vi "Measurement UI.vi"() -> ()   [LabVIEW 2023, in "FPT_Compression UI.lvlib"]
uses:
  FPT_Compression UI.lvlib
panel:
  in  "Measurement Graph":T1(tab)
  out "General Graph 1":T2(graph)
  out "General Graph 2":T2(graph)
  out "General Graph 3":T2(graph)
  out "General Graph 4":T2(graph)
  out "General Graph 5":T2(graph)
  out "PAE@Pin(s)":string[](array[string])
  out "Gain@Pin(s)":string[](array[string])
  out "Pout@Pin(s)":string[](array[string])
  out "Pout@Pin vs Freq":dbl[][](array[numeric])
  out "PAE vs Pin per Freq":dbl[][](array[numeric])
  in  "RFSG attenuation s2p path name":string caption="RFSG ATTENUATION S2P PATH NAME"
  in  "RFmx attenuation s2p path name":string caption="RFmx ATTENUATION S2P PATH NAME"
  in  "RFSG attenuation path name":string caption="RFSG ATTENUATION PATH NAME"
  in  "RFmx attenuation path name":string caption="RFmx ATTENUATION PATH NAME"
  out "Gain vs Pin per Freq":dbl[][](array[numeric])
  out "Group B Graph":refnum<vi>[](array[refnum])
  out "Group A Graph":refnum<vi>[](array[refnum])
  in  "Power sequencing file path":string
  in  "RFSG name":string="5842_0"
  in  "RFSG attenuation mode":T3(ring)=enum."s2p File"
  in  "RFSG s2p file path":string
  in  "RFmx name":string="5842_0"
  in  "RFmx attenuation mode":T3(ring)=enum."Constant Attenuation"
  in  "RFmx s2p file path":string
  out "All Graph Refs":refnum<vi>[](array[refnum])
  out "Pout vs Pin per Freq":dbl[][](array[numeric])
  out "OPxdB vs Freq":dbl[][](array[numeric])
  out "Linear Gain vs Freq":dbl[][](array[numeric])
  out "Frequencies":string[](array[string])
  out "OPxdB(s)":string[](array[string])
  out "Linear Gain(s)":string[](array[string])
  out "Full Data per Frequency":string[][](array[string])
  out "Pin(s)":string[](array[string])
  in  "Compression_Stimulus Mode":T4(ring)
  in  "SMU name":string caption="SMU Name"
  out "Table 2 Header":string[](array[string])
  out "Table 1 Header":string[](array[string])
  out "Gain@Pin vs Freq":dbl[][](array[numeric])
  out "PAE@Pin vs Freq":dbl[][](array[numeric])
  in  "Power sequencing file validity check":bool
  out "MeasTable 1":string[][](table)
  out "MeasTable 2":string[][](table)
  in  "Mode of operation":T5(ring) caption="Configuration"
  in  "Tab Control":T6(tab)
  in  "Power sequencing file path_update":path caption="Power Sequencing File Path"
  in  "SMU channel":string caption="SMU Channel"
  in  "SMU name_update":refnum<k15> caption="SMU Name"
  in  "RFmx port":string(combo)="port2" caption="RFmx Port"
  in  "RFSG port":string(combo)="port1" caption="RFSG Port"
  in  "RFSG name_update":refnum<k15> caption="RFSG Name"
  in  "RFSG attenuation mode_tab":T3(tab)=enum."s2p File" caption="RFSG Attenuation Mode"
  in  "RFSG external attenuation (dB)":dbl caption="External Attenuation" format="%#.3fdB"
  in  "RFSG s-parameters orientation":enum32{"Port1 Towards DUT", "Port2 Towards DUT"}(ring) caption="Orientation"
  in  "RFSG s2p file path_update":path caption="S2P File Path"
  in  "RFmx attenuation mode_tab":T3(tab)=enum."s2p File" caption="RFmx Attenuation Mode"
  in  "RFmx external attenuation (dB)":dbl caption="External Attenuation" format="%#.3fdB"
  in  "RFmx s2p file path_update":path caption="S2P File Path"
  in  "RFmx s-parameters orientation":enum32{"Port1 Towards DUT", "Port2 Towards DUT"}(ring) caption="Orientation"
  in  "RFmx name_update":refnum<k15> caption="RFmx Name"
  in  "DC & RF Mode":T4(tab)
  in  "CP_CW_DC Source Delay (s)":dbl caption="DC Source Delay" format="%#ps"
  in  "CP_PRF_RFmx Trigger Delay (s)":dbl caption="RFmx Trigger Delay" format="%#ps"
  in  "CP_PRF_PRI (s)":dbl=0.001 caption="PRI" format="%#ps"
  in  "CP_PRF_RF Pulse Width (s)":dbl=0.0001 caption="RF Pulse Width" format="%#ps"
  in  "CP_PRF_DC Source Delay (s)":dbl caption="DC Source Delay" format="%#ps"
  in  "PP_PRF_ON Current Limit (A)":dbl=0.2 caption="Pulse ON Current Limit" format="%#pA"
  in  "PP_PRF_PRI (s)":dbl=0.001 caption="PRI" format="%#ps"
  in  "PP_PRF_RF Pulse Width (s)":dbl=0.0001 caption="RF Pulse Width" format="%#ps"
  in  "PP_PRF_DC Source Delay (s)":dbl caption="DC Source Delay" format="%#ps"
  in  "PP_PRF_RFmx Trigger Delay (s)":dbl caption="RFmx Trigger Delay" format="%#ps"
  in  "PP_PRF_DC Pulse Width (s)":dbl=0.0008 caption="DC Pulse Width" format="%#ps"
  in  "PP_PRF_Bias Voltage Level (V)":dbl caption="Pulse OFF Voltage Level" format="%#pV"
  in  "PP_PRF_Bias Current Limit (A)":dbl=0.2 caption="Pulse OFF Current Limit" format="%#pA"
  in  "Compression_DC Measurement Interval (s)":dbl=5e-05 caption="DC Measurement Interval" format="%#ps"
  in  "Compression_RF Measurement Interval (s)":dbl=5e-05 caption="RF Measurement Interval" format="%#ps"
  in  "Compression_Target Pin (dBm)":dbl=1.0 caption="Target Pin" format="%#pdBm"
  in  "Compression_Expected DUT Gain (dB)":dbl=17.5 caption="Expected DUT Gain" format="%#pdB"
  in  "Compression_Max Linear Range (dBm)":dbl=-10.0 caption="Max Linear Range" format="%#pdBm"
  in  "Compression_Compression Point (dB)":dbl=1.0 caption="PxdB" format="%#pdB"
  in  "Compression_RFSG Frequency Start (Hz)":dbl=6000000000.0 caption="Frequency Start" step=1000000.0 format="%#pHz"
  in  "Compression_RFSG Power Start (dBm)":dbl=-20.0 caption="Power Start" format="%#pdBm"
  in  "Compression_RFSG Power Step Size (dB)":dbl=1.0 caption="Power Step Size" format="%#pdB"
  in  "Compression_RFSG Power Stop(dBm)":dbl=4.0 caption="Power End" format="%#pdBm"
  in  "Compression_RBW (Hz)":dbl=5000000.0 caption="RBW" format="%#pHz"
  in  "Compression_RFSG Frequency Stop (Hz)":dbl=18000000000.0 caption="Frequency Stop" step=1000000.0 format="%#pHz"
  in  "Compression_RFSG Number of Frequency Step":i32=10 caption="Number of Steps"
  out "Status":string
  # "Frequency Sweep"
  # "Power Sweep"
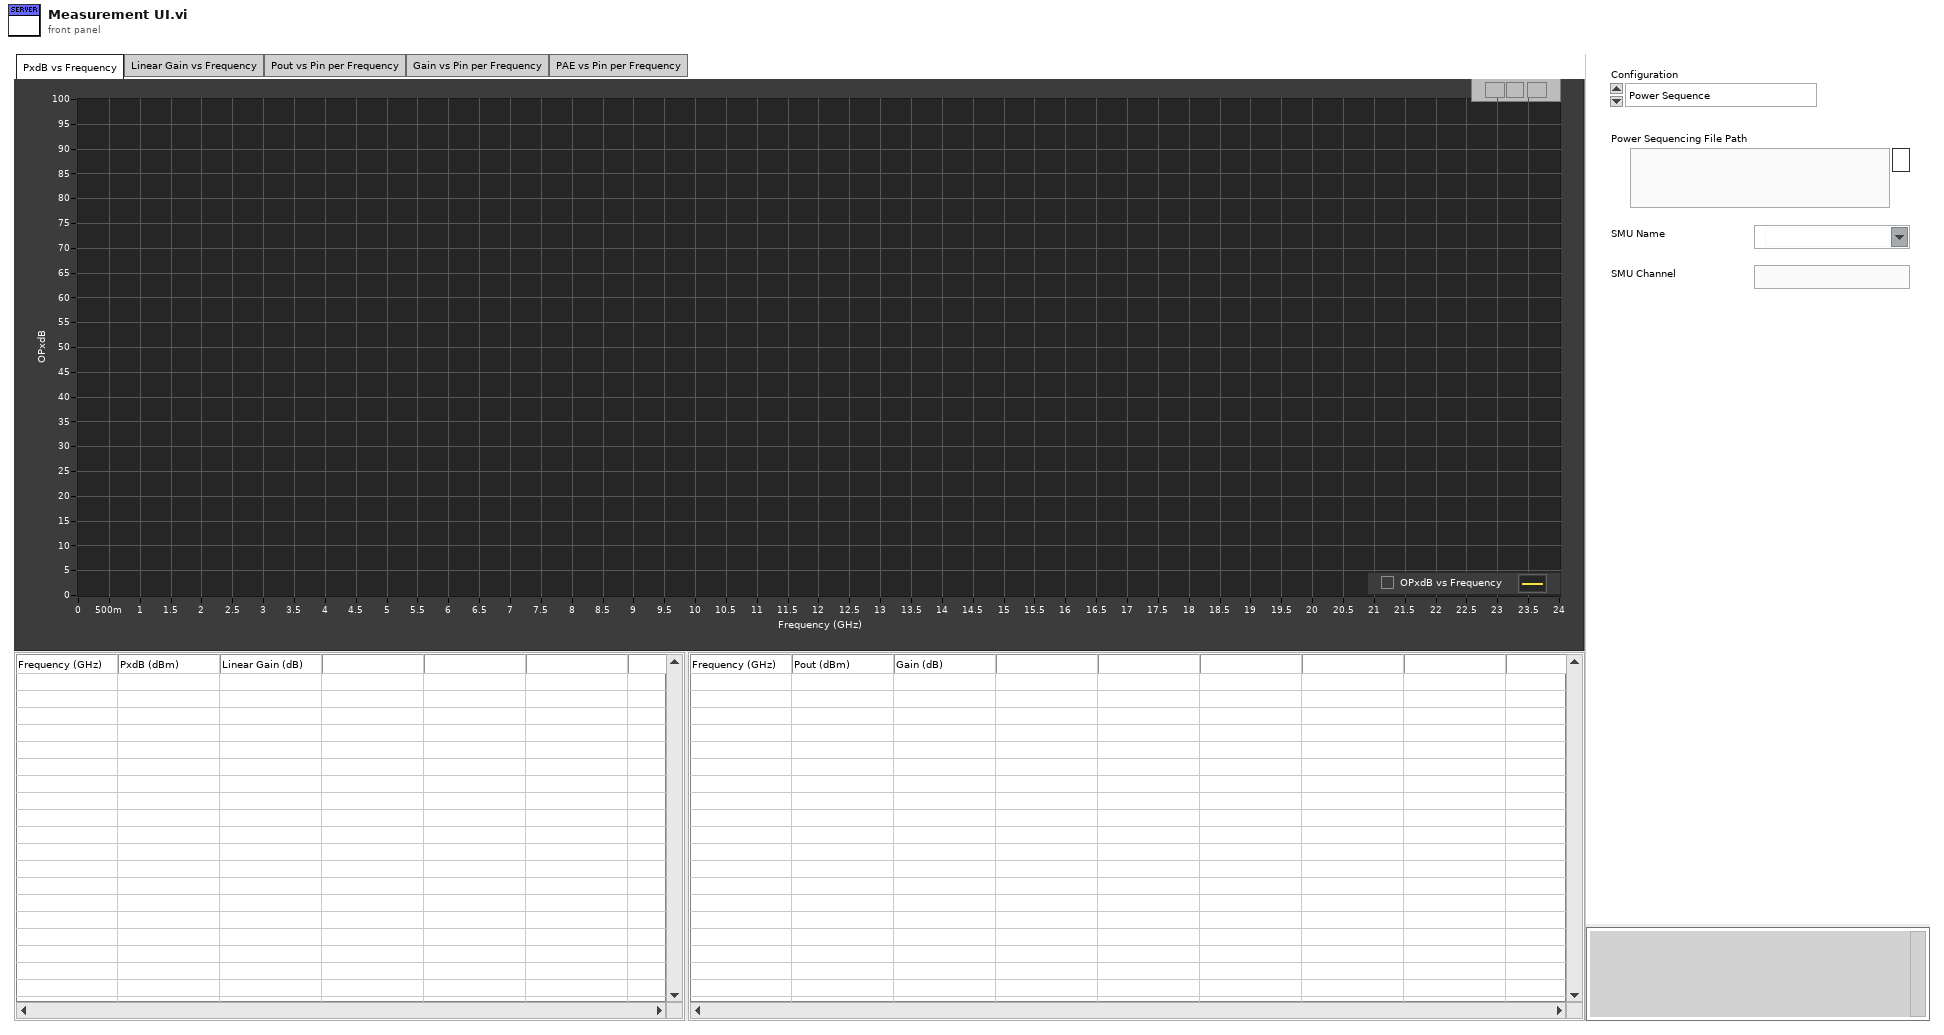
[diagram p1: front panel]
types:
  T1 = enum32{"PxdB vs Frequency", "Linear Gain vs Frequency", "Pout vs Pin per Frequency", "Gain vs Pin per Frequency", "PAE vs Pin per Frequency", "Hidden Controls"}
  T2 = cluster{"Load currents":dbl[], "Efficiency":dbl[]}[]
  T3 = enum32{"<None>", "Constant Attenuation", "s2p File"}
  T4 = enum32{"Constant Power and RF", "Constant Power and Pulsed RF", "Pulsed Power and RF"}
  T5 = enum32{"Power Sequence", "HW + Correction", "Mode", "Measurement 1"}
  T6 = enum32{"Power Sequence", "Correction", "Mode", "Measurement 1"}
  T7 = enum16{"<None>", "Constant Attenuation", "s2p File"}
  T8 = cluster{"Shift":bool, "Ctrl":bool, "Alt":bool, "Cmd":bool, "Opt":bool}
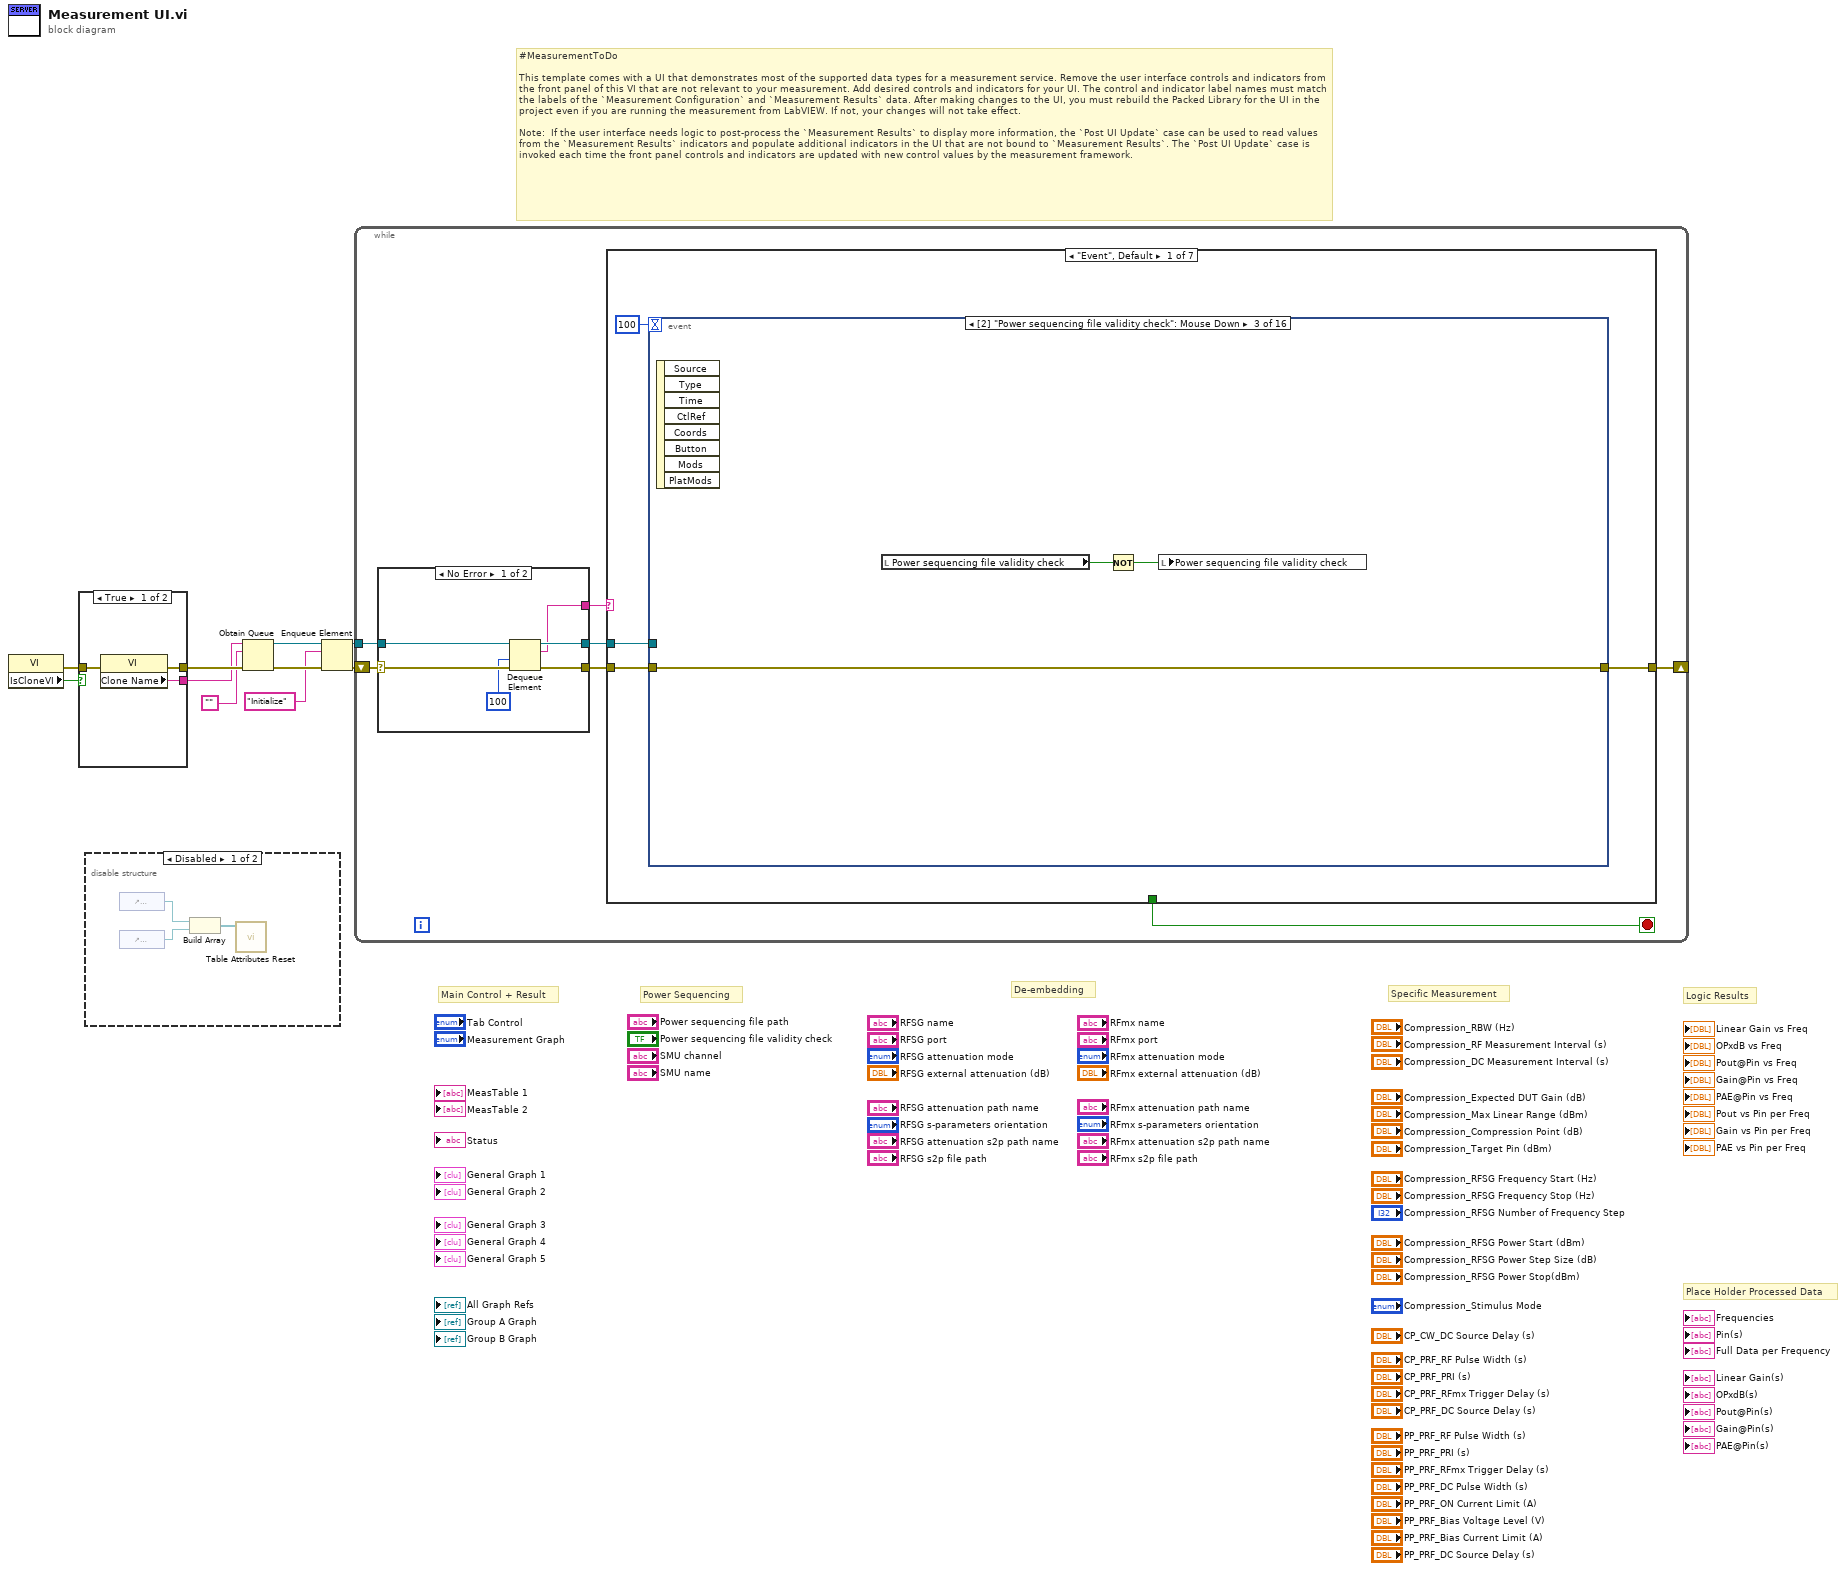
[diagram p0: block diagram]
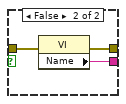
[diagram p3: hidden frame]
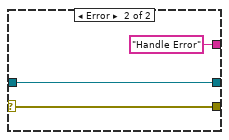
[diagram p4: hidden frame]
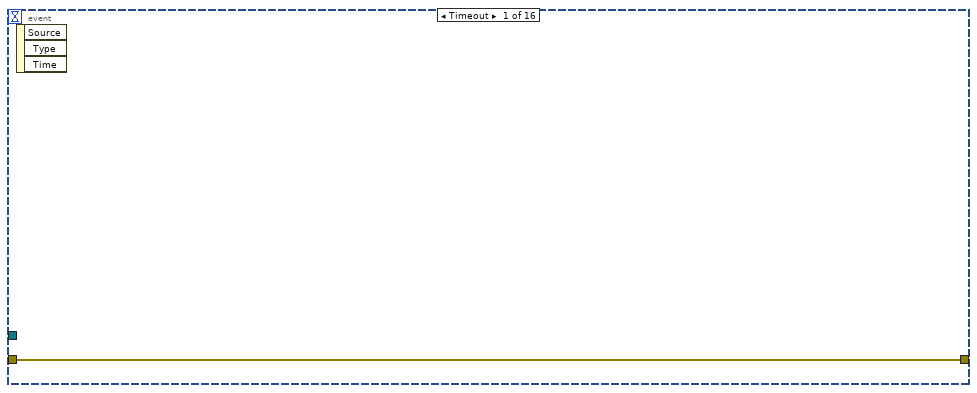
[diagram p5: hidden frame]
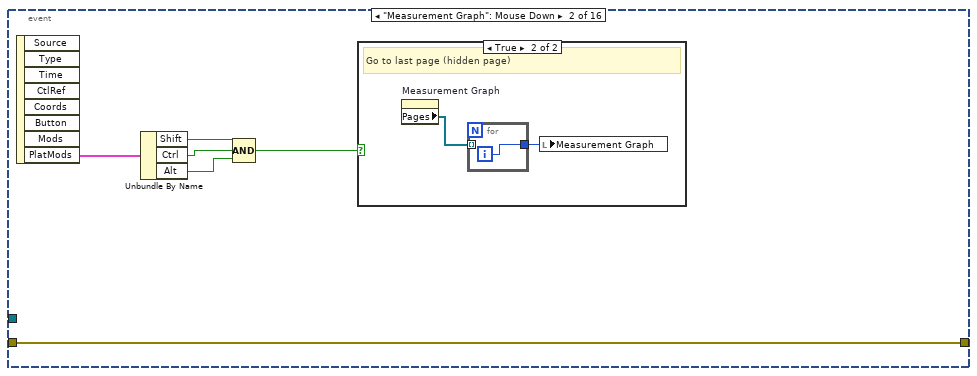
[diagram p6: hidden frame]
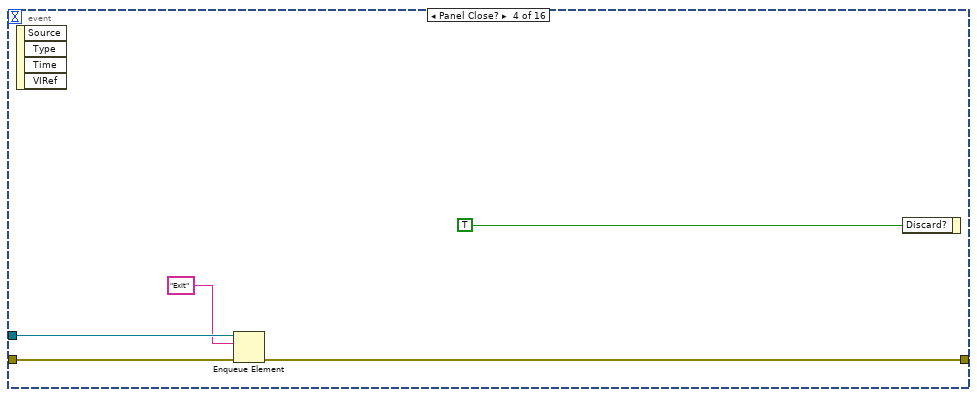
[diagram p8: hidden frame]
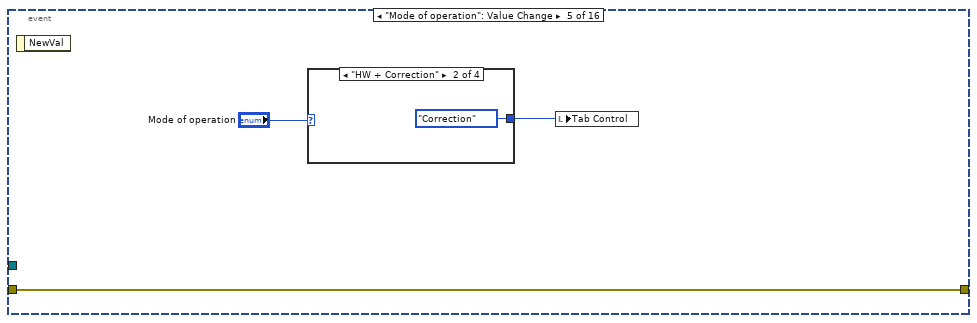
[diagram p9: hidden frame]
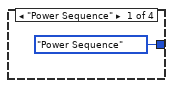
[diagram p10: hidden frame]
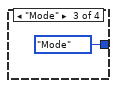
[diagram p11: hidden frame]
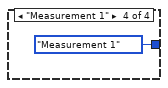
[diagram p12: hidden frame]
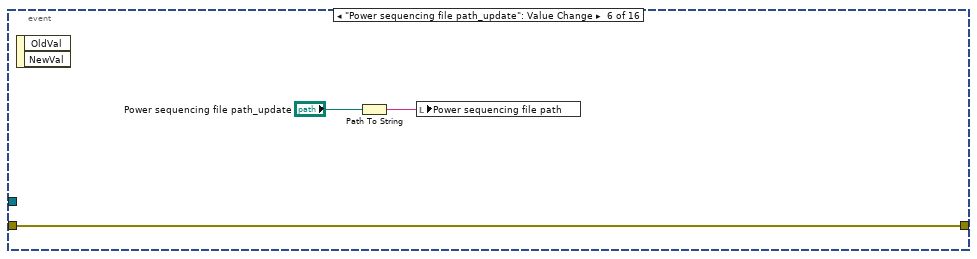
[diagram p13: hidden frame]
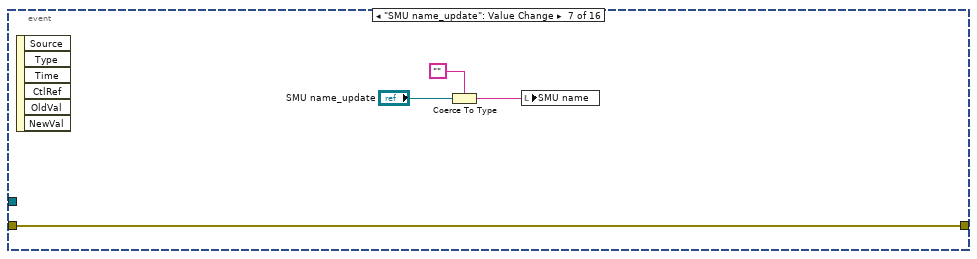
[diagram p14: hidden frame]
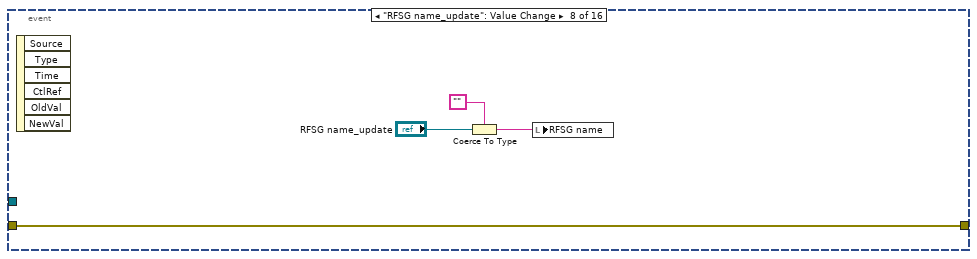
[diagram p15: hidden frame]
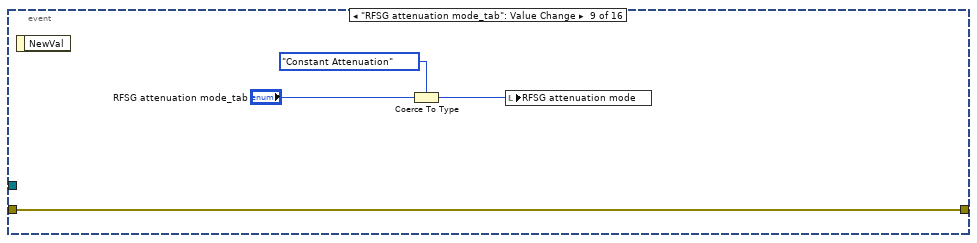
[diagram p16: hidden frame]
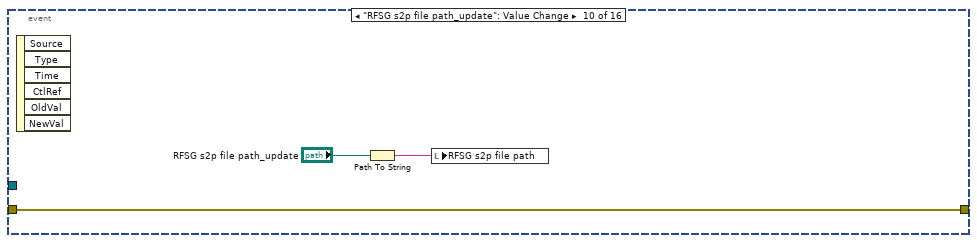
[diagram p17: hidden frame]
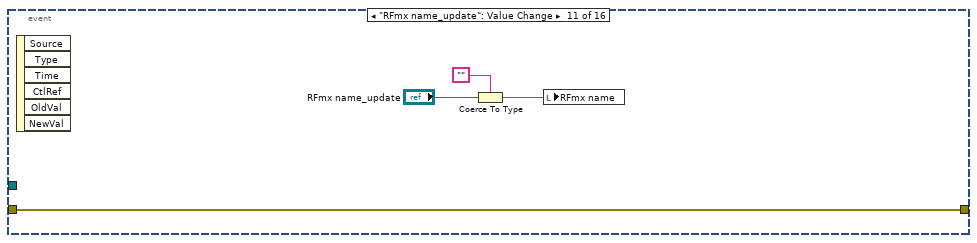
[diagram p18: hidden frame]
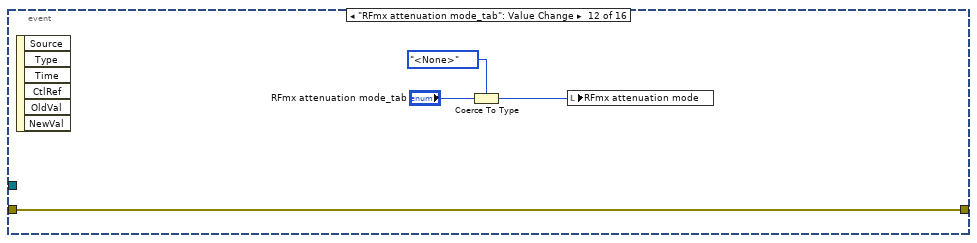
[diagram p19: hidden frame]
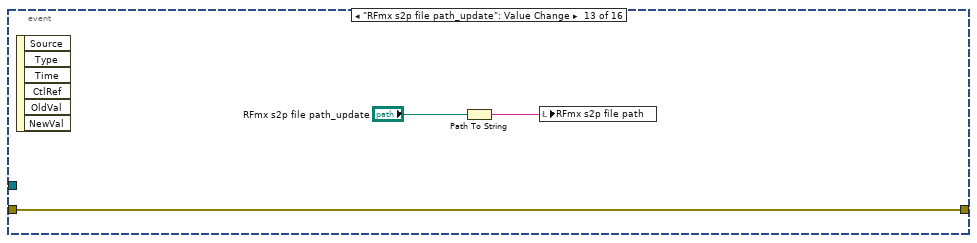
[diagram p20: hidden frame]
diagram:
  # "Logic Results"
  # "Place Holder Processed Data"
  # "Specific Measurement"
  # "De-embedding"
  # "Power Sequencing"
  # "Main Control + Result"
  # "#MeasurementToDo  \n\nThis template comes with a UI that demonstrates most of the supported data types for a measurement service. Remove the user interface controls and indicators from the front panel of this VI that are not relevant to your measurement. Add desired controls and indicators for your UI. The control and indicator label names must match the labels of the `Measurement Configuration` and `Measurement Results` data. After making changes to the UI, you must rebuild the Packed Library for the UI in the project even if you are running the measurement from LabVIEW. If not, your changes will not take effect.\n\nNote:  If the user interface needs logic to post-process the `Measurement Results` to display more information, the `Post UI Update` case can be used to read values from the `Measurement Results` indicators and populate additional indicators in the UI that are not bound to `Measurement Results`. The `Post UI Update` case is invoked each time the front panel controls and indicators are updated with new control values by the measurement framework."
  n1 = property class="VI"() -> (error out=w1:errorcluster, "IsCloneVI"=w2:bool)  [unwired: 2 in, 1 out]
  n2 = case shown="True" w2 {
    tunnel: [w13 w16] -> w10
    tunnel: [w12 w15] -> w9
    tunnel: w1 -> [w11 w14]
    frame True {
      n3 = property class="VI"(error in=w11) -> (error out=w13:errorcluster, "Clone Name"=w12:string)  [unwired: 1 in, 1 out]
    }
    frame False {
      n4 = property class="VI"(error in=w14) -> (error out=w16:errorcluster, "Name"=w15:string)  [unwired: 1 in, 1 out]
    }
  }
  n5 = disable-structure shown="Disabled" {
    frame Disabled {
      n6 = control-ref of="MeasTable 2"() -> (w19:refnum<vi>)
      n7 = control-ref of="MeasTable 1"() -> (w18:refnum<vi>)
      n8 = Build Array(w19, w18) -> (w17:refnum<vi>[])
      n9 = call "Table Attributes Reset.vi"("Table Refs"=w17) -> ()  [unwired: 11 in]
    }
    frame Enabled {
    }
  }
  n10 = Obtain Queue(name (unnamed)=w9, element data type="", error in (no error)=w10) -> (queue out=w6:refnum<queue>, error out=w8:errorcluster)  [unwired: 2 in, 1 out]
  n11 = Enqueue Element(queue=w6, element="Initialize", error in (no error)=w8) -> (queue out=w5:refnum<queue>, error out=w7:errorcluster)  [unwired: 1 in, 1 out]
  n12 = while {
    shift-right: [w21] -> _
    shift-left: w7 -> [w26]
    tunnel: w5 -> [w24]
    stop <- w20 stop-if-true
    n13 = case shown="No Error" w26 {
      selector: w26 -> [w32 w35]
      tunnel: [w31 w35] -> w25
      tunnel: w24 -> [w30 w34]
      tunnel: [w29 w34] -> w23
      tunnel: [w28 "Handle Error"] -> w22
      frame No Error {
        n14 = Dequeue Element(queue=w30, timeout in ms (-1)=100, error in (no error)=w32) -> (queue out=w29:refnum<queue>, element=w28:string, error out=w31:errorcluster)  [unwired: 1 out]
      }
      frame Error {
      }
    }
    n15 = case shown="\"Event\", Default" w22 {
      tunnel: w25 -> [w38 w153 w220 w262 w270 w277 w278]
      tunnel: w23 -> [w36 _ w219 w260 _ w275 _]
      tunnel: [w39 w153 w220 w261 w265 w272 w278] -> w21
      tunnel: [_ _ _ _ _ TRUE _] -> w20
      frame "Event", Default {
        n16 = event shown="[2] \"Power sequencing file validity check\": Mouse Down" {
          selector: _ -> [_ _ _ _ _ _ _ _ _ _ _ _ _ _ _ _]
          dyn-events: _ -> [_ _ _ _ _ _ _ _ _ _ _ _ _ _ _ _]
          timeout: 100 -> [_ _ _ _ _ _ _ _ _ _ _ _ _ _ _ _]
          tunnel: [w40 w41 w52 w55 w59 w65 w71 w72 w76 w80 w83 w87 w91 w97 w110 w131] -> w39
          tunnel: w38 -> [w40 w41 w52 w56 w59 w65 w71 w72 w76 w80 w83 w87 w91 w97 w112 w132]
          tunnel: w36 -> [_ _ _ w54 _ _ _ _ _ _ _ _ _ _ _ _]
          event Timeout {
            n17 = event-data() -> ()  [unwired: 1 in, 3 out]
          }
          event "Measurement Graph": Mouse Down {
            n18 = event-data() -> ("PlatMods"=w46:T8)  [unwired: 1 in, 7 out]
            n19 = Unbundle By Name(w46) -> ("Shift"=w45:bool, "Ctrl"=w44:bool, "Alt"=w43:bool)
            n20 = Compound Arithmetic op=AND(w45, w44, w43) -> (w42:bool)
            n21 = case shown="True" w42 {
              frame False {
              }
              frame True {
                # "Go to last page (hidden page)"
                n22 = property on="Measurement Graph" class="TabCtl (strict)"() -> ("Pages"=w48:refnum<vi>[])  [unwired: 2 in, 2 out]
                n23 = for {
                  tunnel: w48 -> [_] mode=indexing
                  tunnel: [w49] -> w47
                  i -> [w49]
                }
                n24 = local write "Measurement Graph"(w47) -> ()
              }
            }
          }
          event "Power sequencing file validity check": Mouse Down {
            n25 = event-data() -> ()  [unwired: 1 in, 8 out]
            n26 = local read "Power sequencing file validity check"() -> (w51:bool)
            n27 = Not(x=w51) -> (.not. x?=w50:bool)
            n28 = local write "Power sequencing file validity check"(w50) -> ()
          }
          event Panel Close? {
            n29 = event-data() -> ()  [unwired: 1 in, 4 out]
            n30 = Enqueue Element(queue=w54, element="Exit", error in (no error)=w56) -> (error out=w55:errorcluster)  [unwired: 1 in, 2 out]
            n31 = event-data("Discard?"=TRUE) -> ()  [unwired: 1 in, 1 out]
          }
          event "Mode of operation": Value Change {
            n32 = event-data() -> ()  [unwired: 1 in, 1 out]
            n33 = case shown="\"HW + Correction\"" "Mode of operation" {
              tunnel: [T6."Power Sequence" ("Tab Control") T6."Correction" ("Tab Control") T6."Mode" ("Tab Control") T6."Measurement 1" ("Tab Control")] -> w58
              frame "Power Sequence" {
              }
              frame "HW + Correction" {
              }
              frame "Mode" {
              }
              frame "Measurement 1" {
              }
            }
            n34 = local write "Tab Control"(w58) -> ()
          }
          event "Power sequencing file path_update": Value Change {
            n35 = event-data() -> ()  [unwired: 1 in, 2 out]
            n36 = Path To String(path="Power sequencing file path_update") -> (string=w66:string)
            n37 = local write "Power sequencing file path"(w66) -> ()
          }
          event "SMU name_update": Value Change {
            n38 = event-data() -> ()  [unwired: 1 in, 6 out]
            n39 = Coerce To Type(0:"SMU name_update", 1:"") -> (2:w68:string)
            n40 = local write "SMU name"(w68) -> ()
          }
          event "RFSG name_update": Value Change {
            n41 = event-data() -> ()  [unwired: 1 in, 6 out]
            n42 = Coerce To Type(0:"RFSG name_update", 1:"") -> (2:w73:string)
            n43 = local write "RFSG name"(w73) -> ()
          }
          event "RFSG attenuation mode_tab": Value Change {
            n44 = event-data() -> ()  [unwired: 1 in, 1 out]
            n45 = Coerce To Type(0:"RFSG attenuation mode_tab", 1:T3."Constant Attenuation" ("RFSG attenuation mode")) -> (2:w78:T3)
            n46 = local write "RFSG attenuation mode"(w78) -> ()
          }
          event "RFSG s2p file path_update": Value Change {
            n47 = event-data() -> ()  [unwired: 1 in, 6 out]
            n48 = Path To String(path="RFSG s2p file path_update") -> (string=w81:string)
            n49 = local write "RFSG s2p file path"(w81) -> ()
          }
          event "RFmx name_update": Value Change {
            n50 = event-data() -> ()  [unwired: 1 in, 6 out]
            n51 = Coerce To Type(0:"RFmx name_update", 1:"") -> (2:w85:string)
            n52 = local write "RFmx name"(w85) -> ()
          }
          event "RFmx attenuation mode_tab": Value Change {
            n53 = event-data() -> ()  [unwired: 1 in, 6 out]
            n54 = Coerce To Type(0:"RFmx attenuation mode_tab", 1:T7."<None>" ("RFmx attenuation mode")) -> (2:w88:T7)
            n55 = local write "RFmx attenuation mode"(w88) -> ()
          }
          event "RFmx s2p file path_update": Value Change {
            n56 = event-data() -> ()  [unwired: 1 in, 6 out]
            n57 = Path To String(path="RFmx s2p file path_update") -> (string=w92:string)
            n58 = local write "RFmx s2p file path"(w92) -> ()
          }
          event "DC & RF Mode": Value Change {
            n59 = event-data() -> ()  [unwired: 1 in, 6 out]
            n60 = Coerce To Type(0:"DC & RF Mode", 1:T4."Constant Power and RF" ("Compression_Stimulus Mode")) -> (2:w95:T4)
            n61 = local write "Compression_Stimulus Mode"(w95) -> ()
          }
          event "General Graph 1", "General Graph 2": Cursor Move {
            n62 = event-data() -> ("CtlRef"=w103:refnum<vi>, "PointIdx"=w109:i32, "CursLoc"=w107:cluster{"X":dbl, "Y":dbl})  [unwired: 1 in, 6 out]
            n63 = Unbundle By Name(w107) -> ("X"=w106:dbl)
            n64 = property on="Group A Graph" class="Arr (strict)"() -> ("Value"=w104:refnum<vi>[])  [unwired: 2 in, 2 out]
            n65 = Search 1D Array(1D array=w104, element=w103) -> (index of element=w105:i32)  [unwired: 1 in]
            n66 = Delete From Array(array=w104, index=w105) -> (array with subset deleted=w102:refnum<vi>[])  [unwired: 1 in, 1 out]
            n67 = call "Graph Cursor Update.vi"("Action"=enum16{"Reset", "Update"}."Update", "error in"=w112, "New X position"=w106, "Cursor Type"=enum16{"Movable", "Fixed", "All"}."Movable", "Graph Refs in"=w102) -> ("error out"=w111:errorcluster)  [unwired: 5 in, 1 out]
            n68 = control-ref of="MeasTable 1"() -> (w99:refnum<vi>)
            n69 = call "Table Highlight.vi"("Action"=enum16{"Reset", "Highlight 1 Row"}."Highlight 1 Row", "error in"=w111, "Color Box"=u32 16776960, "Row"=w109, "Table Ref in"=w99) -> ("error out"=w110:errorcluster)  [unwired: 5 in, 1 out]
          }
          event "General Graph 3", "General Graph 4", "General Graph 5": Cursor Move {
            # "------------------------Table2------------------------\n<Freq><Pin><Pout><Gain><PAE>"
            n70 = event-data() -> ("CtlRef"=w125:refnum<vi>, "PointIdx"=w115:i32, "CursLoc"=w129:cluster{"X":dbl, "Y":dbl})  [unwired: 1 in, 6 out]
            n71 = Unbundle By Name(w129) -> ("X"=w128:dbl)
            n72 = property on="Group B Graph" class="Arr (strict)"() -> ("Value"=w126:refnum<vi>[])  [unwired: 2 in, 2 out]
            n73 = Search 1D Array(1D array=w126, element=w125) -> (index of element=w127:i32)  [unwired: 1 in]
            n74 = Delete From Array(array=w126, index=w127) -> (array with subset deleted=w124:refnum<vi>[])  [unwired: 1 in, 1 out]
            n75 = call "Graph Cursor Update.vi"("Action"=enum16{"Reset", "Update"}."Update", "error in"=w132, "New X position"=w128, "Cursor Type"=enum16{"Movable", "Fixed", "All"}."Movable", "Graph Refs in"=w124) -> ("error out"=w131:errorcluster)  [unwired: 5 in, 1 out]
            n76 = local read "Frequencies"() -> (w116:string[])
            n77 = local read "Pin(s)"() -> (w119:string[])
            n78 = Index Array(array=w119, index=w115) -> (element=w118:string)
            n79 = local read "Full Data per Frequency"() -> (w120:string[][])
            n80 = local read "Table 2 Header"() -> (w113:string[])
            n81 = for {
              tunnel: [w133] -> w117 mode=indexing
              tunnel: w118 -> [w133]
              tunnel: w116 -> [_] mode=indexing
            }
            n82 = control-ref of="MeasTable 2"() -> (w122:refnum<vi>)
            n83 = call "Get Data per Frequency at Pin Point Index.vi"("Pin Point Index"=w115, "Full Data per Freq"=w120) -> ("Focused Data"=w114:string[][])  [unwired: 9 in]
            n84 = Build Array (concatenate)(w116, w117, w114) -> (w121:string[][])
            n85 = call "Table Set Header Name and Data (String).vi"("Data"=w121, "Header"=w113, "Table Ref"=w122) -> ()  [unwired: 9 in]
          }
        }
      }
      frame "Initialize" {
        w145 = 0
        # "-------Go to Default Page/Tab-------"
        # "-------------------------Assign Graph References in Group-------------------------"
        n86 = local write "Tab Control"(w145) -> ()
        n87 = local write "Mode of operation"(w145) -> ()
        n88 = local write "Measurement Graph"(w145) -> ()
        n89 = control-ref of="General Graph 1"() -> (w148:refnum<vi>)
        n90 = control-ref of="General Graph 2"() -> (w147:refnum<vi>)
        n91 = control-ref of="General Graph 3"() -> (w146:refnum<vi>)
        n92 = control-ref of="General Graph 4"() -> (w137:refnum<vi>)
        n93 = control-ref of="General Graph 5"() -> (w136:refnum<vi>)
        n94 = Build Array(w148, w147, w146, w137, w136) -> (w144:refnum<vi>[])
        n95 = Build Array(w148, w147) -> (w143:refnum<vi>[])
        n96 = Build Array(w146, w137, w136) -> (w138:refnum<vi>[])
        n97 = local write "All Graph Refs"(w144) -> ()
        n98 = local write "Group A Graph"(w143) -> ()
        n99 = call "Graph Set Cursor Mode.vi"("Cursor Mode"=enum32{"Free-Drag", "Single-Plot", "Multi-Plot"}."Single-Plot", "Graph Refs in"=w143) -> ("Graph Refs out"=w149:refnum<vi>[])  [unwired: 8 in, 1 out]
        n100 = call "Graph Set Cursor Mode.vi"("Cursor Mode"=enum32{"Free-Drag", "Single-Plot", "Multi-Plot"}."Multi-Plot", "Graph Refs in"=w138) -> ("Graph Refs out"=w142:refnum<vi>[])  [unwired: 8 in, 1 out]
        n101 = local write "Group B Graph"(w138) -> ()
        n102 = call "Graph Cursor Update.vi"("Action"=enum16{"Reset", "Update"}."Reset", "Cursor Type"=enum16{"Movable", "Fixed", "All"}."All", "Graph Refs in"=w149) -> ()  [unwired: 7 in, 2 out]
        n103 = call "Graph Cursor Update.vi"("Action"=enum16{"Reset", "Update"}."Reset", "Cursor Type"=enum16{"Movable", "Fixed", "All"}."All", "Graph Refs in"=w142) -> ()  [unwired: 7 in, 2 out]
        "Table 2 Header" <- string[] ["Frequency (GHz)", "Pin (dBm)", "Pout (dBm)", "Gain (dB)", "PAE (%)"] ("Header")
        "Table 1 Header" <- string[] ["Frequency (GHz)", "PxdB (dBm)", "Linear Gain (dB)", "Pout@Target Pin", "Gain@Target Pin", "PAE@Target Pin"] ("Header")
      }
      frame "Post UI Update" {
        # "--------------------Get Pout@Pin--------------------"
        # "------------------Get PAE@Pin--------------------"
        # "--------------------Get Gain@Pin--------------------"
        # "------------Get Pout(s) and Gain(s) per Frequency------------"
        # "-------------------------Get Frequencies-------------------------"
        # "------------------Get Linear Gain------------------"
        # "--------------------Get OPxdB--------------------"
        # "--------------------Get Pin(s)--------------------"
        # "This case will be triggered, after framework updates the User interface with result values.\nUsed to update data type def"
        n104 = local read "Power sequencing file path"() -> (w216:string)
        n105 = local read "Compression_Stimulus Mode"() -> (w175:T4)
        n106 = local read "RFSG attenuation mode"() -> (w215:T3)
        n107 = local read "RFmx attenuation mode"() -> (w201:T3)
        n108 = local read "SMU name"() -> (w173:string)
        n109 = local read "RFSG s2p file path"() -> (w208:string)
        n110 = local read "RFmx s2p file path"() -> (w207:string)
        n111 = local read "RFSG name"() -> (w212:string)
        n112 = local read "RFmx name"() -> (w203:string)
        n113 = Enqueue Element(queue=w219, element="Post UI Update 2") -> ()  [unwired: 2 in, 3 out]
        n114 = Coerce To Type(0:w173, 1:refnum<k15> refnum ("RFSG name_update")) -> (2:w171:refnum<k15>)
        n115 = Coerce To Type(0:w175, 1:T4."Constant Power and RF" ("DC & RF Mode")) -> (2:w174:T4)
        n116 = local write "SMU name_update"(w171) -> ()
        n117 = Coerce To Type(0:w215, 1:T3."<None>" ("RFSG attenuation mode_tab")) -> (2:w214:T3)
        n118 = Coerce To Type(0:w203, 1:refnum<k15> refnum ("RFSG name_update")) -> (2:w205:refnum<k15>)
        n119 = String To Path(string=w207) -> (path=w206:path)
        n120 = Coerce To Type(0:w212, 1:refnum<k15> refnum ("RFSG name_update")) -> (2:w210:refnum<k15>)
        n121 = Coerce To Type(0:w201, 1:T3."<None>" ("RFmx attenuation mode_tab")) -> (2:w202:T3)
        n122 = String To Path(string=w216) -> (path=w217:path)
        n123 = String To Path(string=w208) -> (path=w209:path)
        n124 = local write "DC & RF Mode"(w174) -> ()
        n125 = local write "RFmx name_update"(w205) -> ()
        n126 = local write "RFmx attenuation mode_tab"(w202) -> ()
        n127 = local write "RFmx s2p file path_update"(w206) -> ()
        n128 = local write "Power sequencing file path_update"(w217) -> ()
        n129 = local write "RFSG name_update"(w210) -> ()
        n130 = local write "RFSG attenuation mode_tab"(w214) -> ()
        n131 = local write "RFSG s2p file path_update"(w209) -> ()
        n132 = local read "Pout vs Pin per Freq"() -> (w196:dbl[][])
        n133 = local read "Linear Gain vs Freq"() -> (w190:dbl[][])
        n134 = local read "OPxdB vs Freq"() -> (w192:dbl[][])
        n135 = Index Array(array=w196) -> (element=w195:dbl[])  [unwired: 2 in]
        n136 = Index Array(array=w192, index (row)=1) -> (element=w189:dbl[])  [unwired: 1 in]
        n137 = Index Array(array=w190, index (row)=1) -> (element=w187:dbl[])  [unwired: 1 in]
        n138 = local read "Gain vs Pin per Freq"() -> (w181:dbl[][])
        n139 = local read "PAE vs Pin per Freq"() -> (w167:dbl[][])
        n140 = local read "Pout vs Pin per Freq"() -> (w180:dbl[][])
        n141 = Number To Fractional String(number=w195) -> (F-format string=w194:string[])  [unwired: 3 in]
        n142 = Number To Fractional String(number=w189) -> (F-format string=w188:string[])  [unwired: 3 in]
        n143 = Number To Fractional String(number=w187) -> (F-format string=w186:string[])  [unwired: 3 in]
        n144 = local write "Pin(s)"(w194) -> ()
        n145 = local write "OPxdB(s)"(w188) -> ()
        n146 = local write "Linear Gain(s)"(w186) -> ()
        n147 = Delete From Array(array=w180, length=1, index (row)=0) -> (array with subset deleted=w182:dbl[][])  [unwired: 1 in, 1 out]
        n148 = Delete From Array(array=w181, length=1, index (row)=0) -> (array with subset deleted=w183:dbl[][])  [unwired: 1 in, 1 out]
        n149 = Delete From Array(array=w167, length=1, index (row)=0) -> (array with subset deleted=w166:dbl[][])  [unwired: 1 in, 1 out]
        n150 = local read "Linear Gain vs Freq"() -> (w199:dbl[][])
        n151 = Build Array (concatenate)(w182, w183, w166) -> (w184:dbl[][])
        n152 = local read "Pout@Pin vs Freq"() -> (w156:dbl[][])
        n153 = local read "Gain@Pin vs Freq"() -> (w159:dbl[][])
        n154 = local read "PAE@Pin vs Freq"() -> (w161:dbl[][])
        n155 = Number To Fractional String(number=w184) -> (F-format string=w185:string[][])  [unwired: 3 in]
        n156 = local write "Full Data per Frequency"(w185) -> ()
        n157 = Index Array(array=w199) -> (element=w198:dbl[])  [unwired: 2 in]
        n158 = for {
          tunnel: w198 -> [w223] mode=indexing
          tunnel: [w221] -> w197 mode=indexing
          # "Get Plot Names"
          n159 = Format Into String(format string="%.3fGHz", w223) -> (resulting string=w221:string)  [unwired: 2 in, 1 out]
        }
        n160 = Index Array(array=w156, index (row)=1) -> (element=w155:dbl[])  [unwired: 1 in]
        n161 = Index Array(array=w159, index (row)=1) -> (element=w162:dbl[])  [unwired: 1 in]
        n162 = Index Array(array=w161, index (row)=1) -> (element=w164:dbl[])  [unwired: 1 in]
        n163 = Number To Fractional String(number=w155) -> (F-format string=w154:string[])  [unwired: 3 in]
        n164 = Number To Fractional String(number=w162) -> (F-format string=w163:string[])  [unwired: 3 in]
        n165 = Number To Fractional String(number=w164) -> (F-format string=w165:string[])  [unwired: 3 in]
        n166 = local write "Pout@Pin(s)"(w154) -> ()
        n167 = local write "Gain@Pin(s)"(w163) -> ()
        n168 = local write "PAE@Pin(s)"(w165) -> ()
        n169 = local write "Frequencies"(w197) -> ()
      }
      frame "Post UI Update 2" {
        # "---------------Graph5---------------\nPAE vs Pin per Frequency"
        # "---------------Graph2---------------\nLinear Gain vs Frequency"
        # "---------------Graph1---------------\nOPxdB vs Frequency"
        # "---------------Graph4---------------\nGain vs Pin per Frequency"
        # "---------------Graph3---------------\nPout vs Pin per Frequency"
        # "------------------------Table1------------------------\nPout, Gain vs Pin per Freq Graph"
        # "------------------------Table2------------------------\n<Freq><Pin><Pout><Gain><PAE>"
        # "Table1: OPxdB, Gain vs Freq"
        # "Run after Post UI Update. Can be duplicate is need more processing.\nUtilize this case to convert the result to graph or table"
        n170 = local read "Linear Gain vs Freq"() -> (w248:dbl[][])
        n171 = local read "OPxdB vs Freq"() -> (w250:dbl[][])
        n172 = control-ref of="General Graph 1"() -> (w251:refnum<vi>)
        n173 = control-ref of="General Graph 2"() -> (w249:refnum<vi>)
        n174 = Enqueue Element(queue=w260, element="Post UI Update 3", error in (no error)=w262) -> (error out=w261:errorcluster)  [unwired: 1 in, 2 out]
        n175 = call "Graph Assign Plot Names and Data.vi"("Legend Number of Rows"=1, "X Ys Data"=w250, "Graph Ref in"=w251) -> ()  [unwired: 6 in, 3 out]
        n176 = call "Graph Assign Plot Names and Data.vi"("Legend Number of Rows"=1, "X Ys Data"=w248, "Graph Ref in"=w249) -> ()  [unwired: 6 in, 3 out]
        n177 = local read "Table 1 Header"() -> (w227:string[])
        n178 = local read "Linear Gain(s)"() -> (w242:string[])
        n179 = local read "Frequencies"() -> (w244:string[])
        n180 = local read "Pout@Pin(s)"() -> (w226:string[])
        n181 = local read "Gain@Pin(s)"() -> (w225:string[])
        n182 = local read "Pout vs Pin per Freq"() -> (w241:dbl[][])
        n183 = local read "PAE@Pin(s)"() -> (w224:string[])
        n184 = local read "Gain vs Pin per Freq"() -> (w255:dbl[][])
        n185 = local read "OPxdB(s)"() -> (w243:string[])
        n186 = local read "Frequencies"() -> (w235:string[])
        n187 = local read "Frequencies"() -> (w234:string[])
        n188 = control-ref of="MeasTable 1"() -> (w252:refnum<vi>)
        n189 = control-ref of="General Graph 3"() -> (w259:refnum<vi>)
        n190 = control-ref of="General Graph 4"() -> (w256:refnum<vi>)
        n191 = Build Array(w244, w243, w242, w226, w225, w224) -> (w245:string[][])
        n192 = call "Graph Assign Plot Names and Data.vi"("Legend Number of Rows"=5, "X Ys Data"=w241, "Plot Names"=w235, "Graph Ref in"=w259) -> ()  [unwired: 5 in, 3 out]
        n193 = call "Graph Assign Plot Names and Data.vi"("Legend Number of Rows"=5, "X Ys Data"=w255, "Plot Names"=w234, "Graph Ref in"=w256) -> ()  [unwired: 5 in, 3 out]
        n194 = call "Table Set Header Name and Data (String).vi"("Data"=w245, "Header"=w227, "Table Ref"=w252) -> ()  [unwired: 9 in]
        n195 = local read "PAE vs Pin per Freq"() -> (w232:dbl[][])
        n196 = local read "Frequencies"() -> (w233:string[])
        n197 = control-ref of="General Graph 5"() -> (w230:refnum<vi>)
        n198 = call "Graph Assign Plot Names and Data.vi"("Legend Number of Rows"=5, "X Ys Data"=w232, "Plot Names"=w233, "Graph Ref in"=w230) -> ()  [unwired: 5 in, 3 out]
        n199 = local read "Frequencies"() -> (w236:string[])
        n200 = local read "Pin(s)"() -> (w239:string[])
        n201 = Index Array(array=w239) -> (element=w238:string)  [unwired: 1 in]
        n202 = local read "Full Data per Frequency"() -> (w240:string[][])
        n203 = local read "Table 2 Header"() -> (w228:string[])
        n204 = for {
          tunnel: [w264] -> w237 mode=indexing
          tunnel: w238 -> [w264]
          tunnel: w236 -> [_] mode=indexing
        }
        n205 = control-ref of="MeasTable 2"() -> (w254:refnum<vi>)
        n206 = call "Get Data per Frequency at Pin Point Index.vi"("Full Data per Freq"=w240) -> ("Focused Data"=w229:string[][])  [unwired: 10 in]
        n207 = Build Array (concatenate)(w236, w237, w229) -> (w253:string[][])
        n208 = call "Table Set Header Name and Data (String).vi"("Data"=w253, "Header"=w228, "Table Ref"=w254) -> ()  [unwired: 9 in]
      }
      frame "Post UI Update 3" {
        n209 = property on="All Graph Refs" class="Arr (strict)"() -> ("Value"=w269:refnum<vi>[])  [unwired: 2 in, 2 out]
        n210 = call "Graph Cursor Update.vi"("Action"=enum16{"Reset", "Update"}."Update", "error in"=w270, "New X position"=0.0, "Cursor Type"=enum16{"Movable", "Fixed", "All"}."Movable", "Graph Refs in"=w269) -> ("error out"=w265:errorcluster)  [unwired: 5 in, 1 out]
      }
      frame "Exit" {
        # "This case is triggered to close the User Interface from framework"
        n211 = Flush Queue(queue=w275, error in (no error)=w277) -> (queue out=w274:refnum<queue>, error out=w273:errorcluster)  [unwired: 1 out]
        n212 = Release Queue(queue=w274, force destroy? (F)=TRUE, error in (no error)=w273) -> (error out=w272:errorcluster)  [unwired: 2 out]
      }
      frame "Handle Error" {
      }
    }
  }
